vi "Open Project Reference.vi"(8 "error in":errorcluster, 10 "Path":path, 11 "Project Manager in":refnum<class "Project Manager.lvclass">) -> (0 "error out":errorcluster, 3 "Project Manager out":refnum<class "Project Manager.lvclass">)   [LabVIEW 2026, in "Project Manager.lvclass"]
doc: "Open project reference."
uses:
  Project Manager.lvclass
  Project Manager.lvclass/Project Manager.ctl
  Interfaces/ILogger/ILogger Messages/Log Msg/Log Msg.lvclass/Log Msg.ctl
  <vilib>/ActorFramework/Message Enqueuer/Message Enqueuer.lvclass/Message Enqueuer.ctl
  <vilib>/ActorFramework/Message Enqueuer/Enqueue.vi
  Interfaces/ILogger/ILogger Messages/Log Msg/Log Msg.lvclass
  <vilib>/ActorFramework/Message Priority Queue/Priority Enqueue.vi
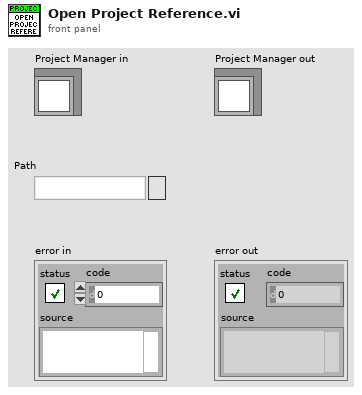
[diagram p1: front panel]
types:
  T1 = typedef "Log Entry--cluster.ctl" = cluster{"Time":timestamp, "Message":string}
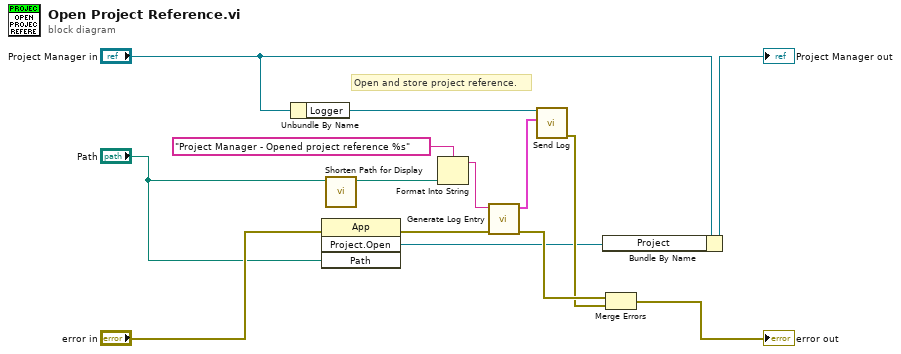
[diagram p0: block diagram]
diagram:
  # "Open and store project reference."
  n1 = Unbundle By Name("Project Manager in") -> ("Logger"=w6:refnum<class "Message Enqueuer.lvclass">)
  n2 = invoke class="App" method="Project.Open"(error in="error in", "Path"="Path") -> (error out=w12:errorcluster, "Project:Open"=w8:refnum<vi>)  [unwired: 2 in, 2 out]
  n3 = call "Shorten Path for Display.vi"("Path"="Path") -> ("Shortened Path"=w3:path)  [unwired: 10 in]
  n4 = Format Into String(format string="Project Manager - Opened project reference %s", w3) -> (resulting string=w2:string)  [unwired: 2 in, 1 out]
  n5 = call "Generate Log Entry.vi"("error in"=w12, "Message"=w2) -> ("error out"=w13:errorcluster, "Log Entry"=w1:T1)  [unwired: 8 in]
  n6 = call "Send Log.vi"("Log Entry"=w1, "Message Enqueuer"=w6) -> ("error out"=w10:errorcluster)  [unwired: 8 in, 1 out]
  n7 = Bundle By Name(cluster="Project Manager in", "Project"=w8) -> (→"Project Manager out":refnum<class "Project Manager.lvclass">)
  n8 = Merge Errors(w13, w10) -> (→"error out":errorcluster)
